vi "WaveAnalysis.vi"() -> (0 "输出图片":picture caption="新图片", 3 "Pixel_in":u8[](array[numeric]) format="%02x", 5 "Gray_in":u8[](array[numeric])=[12, 12, 0, 12, 12, 0, 16, 16, 0, 20, 20, 0, 24, 24, 0, 28, 28, 0, 32, 32, 0, 36, 36, 0, 40, 40, 0, 44, 44, 0, 48, 48, 0, 52, 52, 0, 56, 56, 0, 60, 60, 0, 64, 64, 0, 68, 68, 0, 72, 72, 0, 72, 72, 0, 76, 76, 0, 80, 80, 0, 84, 84, 0, 88, 88, 0, 92, 92, 0, 96, 96, 0, 100, 100, 0, 104, 104, 0, 108, 108, 0, 112, 112, 0, 116, 116, 0, 120, 120, 0, 124, 124, 0, 128, 128, 0, 132, 132, 0, 136, 136, 0, 136, 136, 0, 140, 140, 0, 144, 144, 0, 148, 148, 0, 152, 152, 0, 156, 156, 0, 160, 160, 0, 164, 164, 0, 168, 168, 0, 172, 172, 0, 176, 176, 0, 180, 180, 0, 184, 184, 0, 188, 188, 0, 192, 192, 0, 196, 196, 0, 200, 200, 0, 200, 200, 0, 204, 204, 0, 208, 208, 0, 212, 212, 0, 216, 216, 0, 220, 220, 0, 224, 224, 0, 228, 228, 0, 232, 232, 0, 236, 236, 0, 240, 240, 0, 244, 244, 0, 248, 248, 0, 0, 12, 12, 0, 12, 12, 0, 16, 16, 0, 20, 20, 0, 24, 24, 0, 28, 28, 0, 32, 32, 0, 36, 36, 0, 40, 40, 0, 44, 44, 0, 48, 48, 0, 52, 52, 0, 56, 56, 0, 60, 60, 0, 64, 64, 0, 68, 68, 0, 72, 72, 0, 72, 72, 0, 76, 76, 0, 80, 80, 0, 84, 84, 0, 88, 88, 0, 92, 92, 0, 96, 96, 0, 100, 100, 0, 104, 104, 0, 108, 108, 0, 112, 112, 0, 116, 116, 0, 120, 120, 0, 124, 124, 0, 128, 128, 0, 132, 132, 0, 136, 136, 0, 136, 136, 0, 140, 140, 0, 144, 144, 0, 148, 148, 0, 152, 152, 0, 156, 156, 0, 160, 160, 0, 164, 164, 0, 168, 168, 0, 172, 172, 0, 176, 176, 0, 180, 180, 0, 184, 184, 0, 188, 188, 0, 192, 192, 0, 196, 196, 0, 200, 200, 0, 200, 200, 0, 204, 204, 0, 208, 208, 0, 212, 212, 0, 216, 216, 0, 220, 220, 0, 224, 224, 0, 228, 228, 0, 232, 232, 0, 236, 236, 0, 240, 240, 0, 244, 244, 0, 248, 248] format="%02x")   [LabVIEW 2015]
uses:
  <vilib>/picture/picture.llb/Draw True-Color Pixmap.vi
panel:
  out "像素加粗":picture caption="新图片"
  out "图片缩放":picture caption="新图片"
  in  "像素表路径":path=path "E:/JL-Project/LabView-Project/UPO-Pixel.dat"
  in  "宽度":u32=700
  in  "高度":u32=400
  in  "灰度表路径":path=path "E:/JL-Project/LabView-Project/GrayTable.dat"
  in  "szPixel":u32=3
  in  "m_nGrayScale":u32=64
  in  "m_nCHs":u32=4
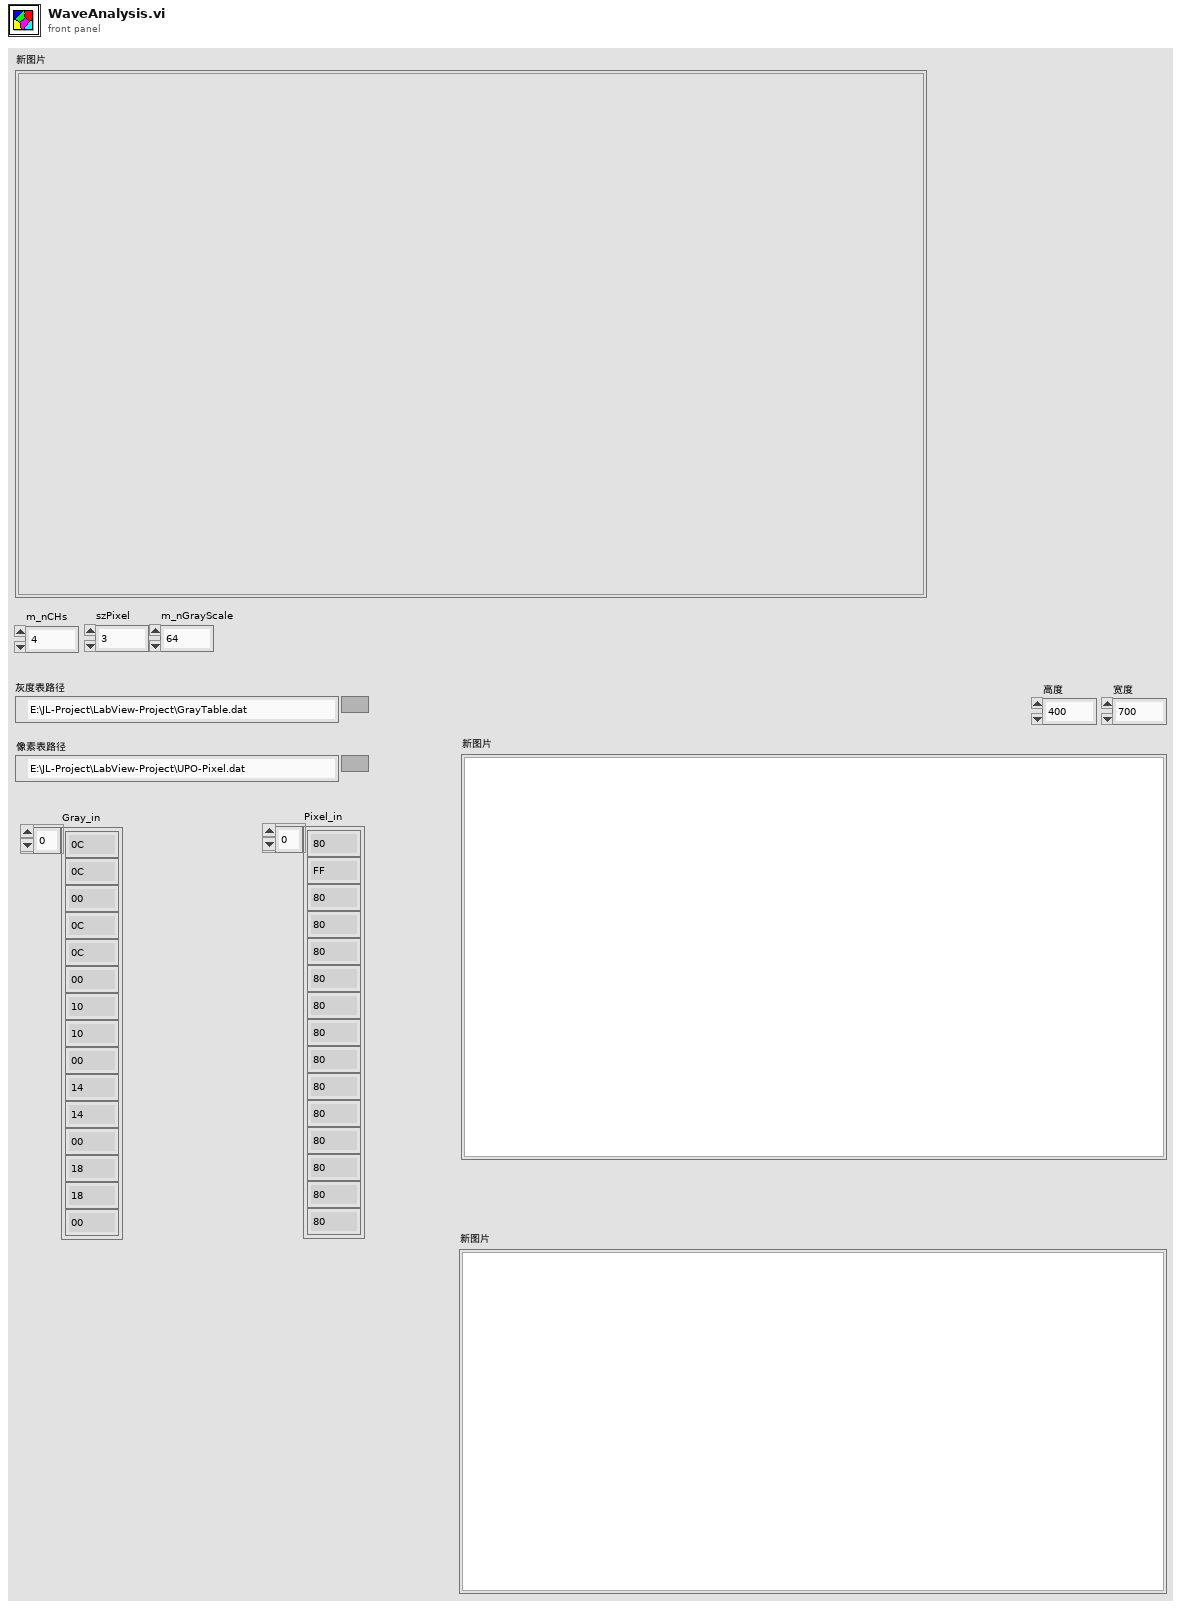
[diagram p1: front panel]
types:
  T1 = enum16{"open", "replace", "create", "open or create", "replace or create", "replace or create with confirmation"}
  T2 = enum16{"big-endian, network order", "native, host order", "little-endian"}
  T3 = typedef "imagedata.ctl" = cluster{"image type":i32, "image depth":i32, "image":u8[], "mask":u8[], "colors":u32[], "Rectangle":cluster{"left":i16, "top":i16, "right":i16, "bottom":i16}}
  T4 = typedef "LVBoundsTypeDef.ctl" = cluster{"Width":u32, "Height":u32}
  T5 = cluster{"left":i16, "top":i16, "right":i16, "bottom":i16}
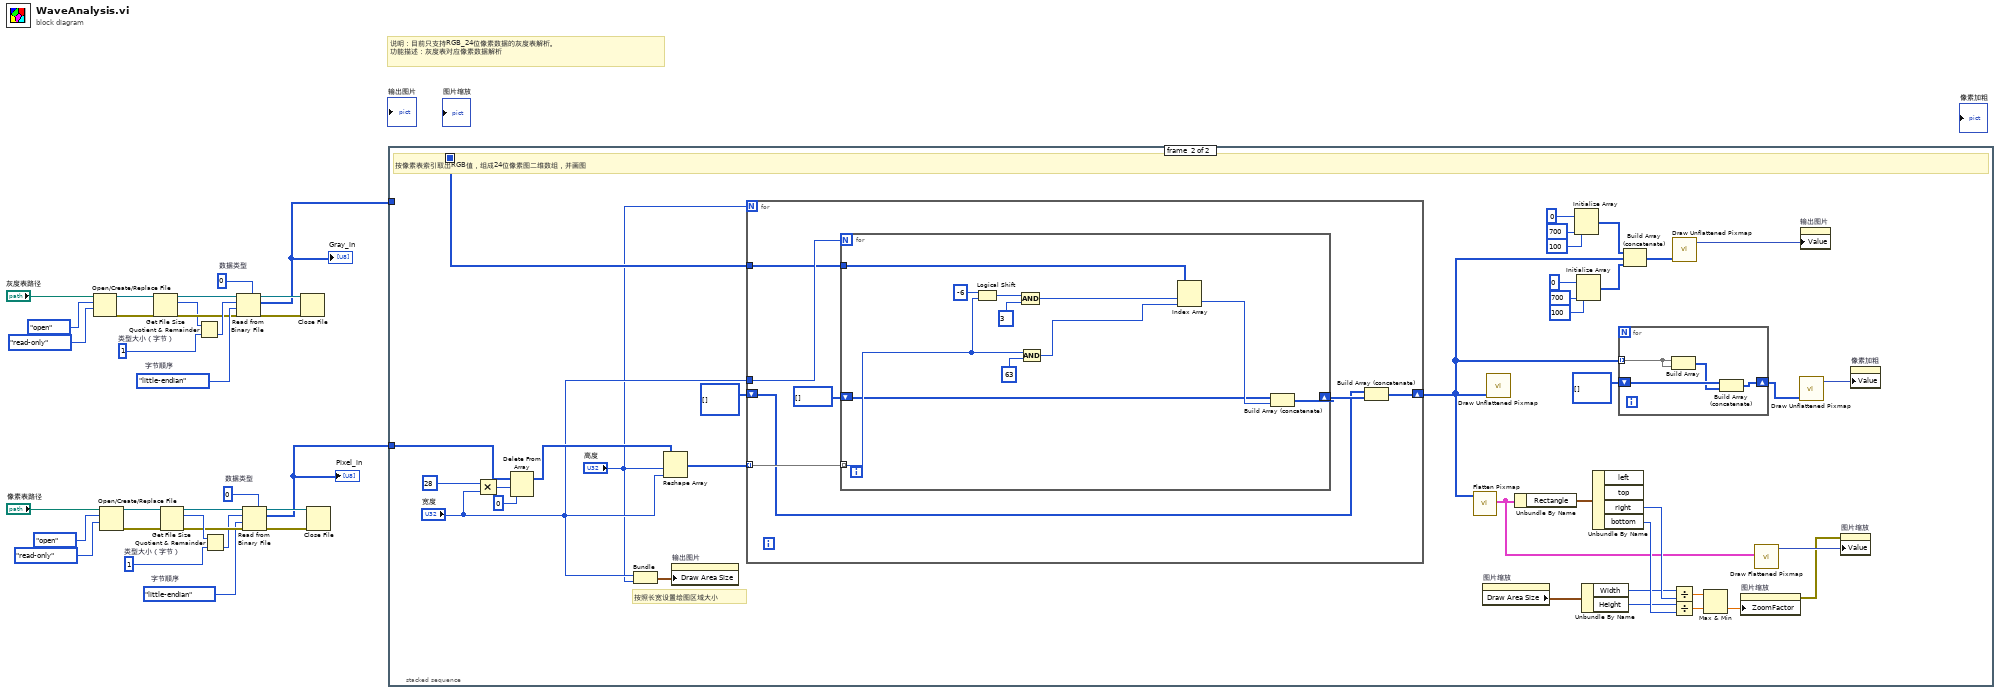
[diagram p0: block diagram]
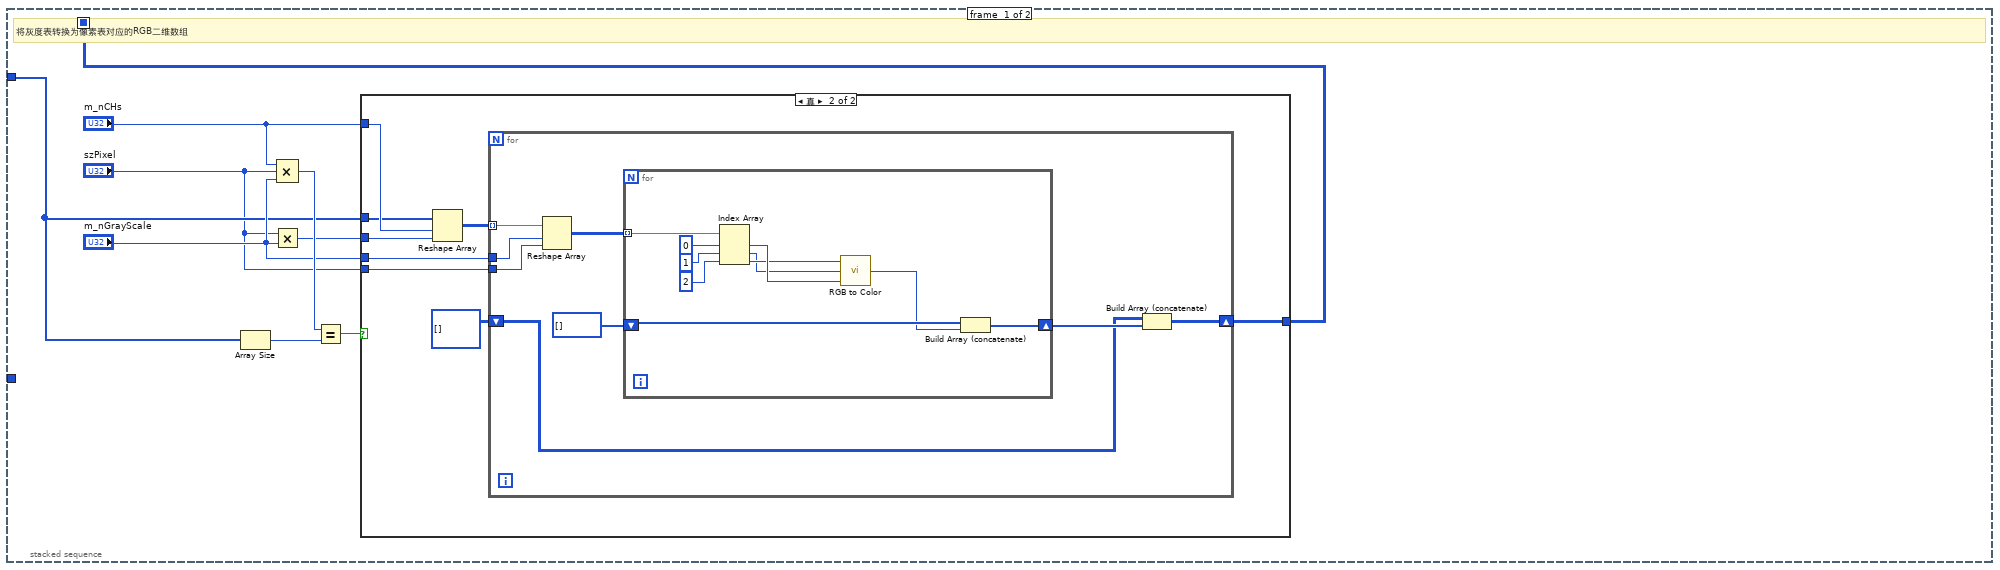
[diagram p2: hidden frame]
diagram:
  w12 = T2."little-endian"  # 字节顺序
  w10 = i64 1  # 类型大小（字节）
  w9 = u8 0  # 数据类型
  w21 = T2."little-endian"  # 字节顺序
  w23 = i64 1  # 类型大小（字节）
  w24 = u8 0  # 数据类型
  # "说明：目前只支持RGB_24位像素数据的灰度表解析。\n功能描述：灰度表对应像素数据解析"
  n1 = Open/Create/Replace File(file path (use dialog)="灰度表路径", operation (0:open)=T1."open", access (0:read/write)=enum16{"read/write", "read-only", "write-only"}."read-only") -> (refnum out=w15:refnum<file>, error out=w14:errorcluster)  [unwired: 3 in, 1 out]
  n2 = Open/Create/Replace File(file path (use dialog)="像素表路径", operation (0:open)=T1."open", access (0:read/write)=enum16{"read/write", "read-only", "write-only"}."read-only") -> (refnum out=w18:refnum<file>, error out=w19:errorcluster)  [unwired: 3 in, 1 out]
  n3 = Get File Size(file=w15, error in=w14) -> (refnum out=w3:refnum<file>, size (in bytes)=w6:i64, 0:w7:errorcluster)
  n4 = Get File Size(file=w18, error in=w19) -> (refnum out=w30:refnum<file>, size (in bytes)=w27:i64, 0:w26:errorcluster)
  n5 = Quotient & Remainder(x=w6, y=w10) -> (floor(x/y)=w11:i64)  [unwired: 1 out]
  n6 = Quotient & Remainder(x=w27, y=w23) -> (floor(x/y)=w22:i64)  [unwired: 1 out]
  n7 = Read from Binary File(5:w9, 8:w7, 9:w12, 10:w11, 11:w3) -> (0:w5:errorcluster, 2:w1:u8[], 3:w4:refnum<file>)  [unwired: 1 in, 1 out]
  "Gray_in" <- w1
  n8 = Read from Binary File(5:w24, 8:w26, 9:w21, 10:w22, 11:w30) -> (0:w28:errorcluster, 2:w2:u8[], 3:w29:refnum<file>)  [unwired: 1 in, 1 out]
  "Pixel_in" <- w2
  n9 = Close File(refnum=w4, error in=w5) -> ()  [unwired: 2 out]
  n10 = Close File(refnum=w29, error in=w28) -> ()  [unwired: 2 out]
  n11 = stacked-sequence {
    seq-local: [w31 _] -> [_ w97]
    tunnel: w1 -> [w33 _]
    tunnel: w2 -> [_ w99]
    frame #0 {
      # "将灰度表转换为像素表对应的RGB二维数组"
      n12 = Array Size(array=w33) -> (size(s)=w38:i32)
      n13 = Multiply(x="szPixel", y="m_nGrayScale") -> (x*y=w35:u32)
      n14 = Compound Arithmetic op=MULTIPLY("m_nCHs", "szPixel", "m_nGrayScale") -> (w39:u32)
      n15 = Equal?(x=w39, y=w38) -> (x = y?=w37:bool)
      n16 = case shown="真" w37 {
        tunnel: "m_nCHs" -> [_ w47]
        tunnel: w33 -> [_ w46]
        tunnel: w35 -> [_ w45]
        tunnel: "szPixel" -> [_ w43]
        tunnel: "m_nGrayScale" -> [_ w42]
        tunnel: [_ w40] -> w31
        frame False {
        }
        frame True {
          n17 = Reshape Array(w46, w47, w45) -> (w44:u8[][])
          n18 = for {
            tunnel: w44 -> [w55] mode=indexing
            tunnel: w43 -> [w53]
            tunnel: w42 -> [w54]
            shift-right: [w49] -> w40
            shift-left: u32[][] [] -> [w50]
            n19 = Reshape Array(w55, w54, w53) -> (w52:u8[][])
            n20 = for {
              tunnel: w52 -> [w63] mode=indexing
              shift-right: [w64] -> w51
              shift-left: u32[] [] -> [w65]
              n21 = Index Array(array=w63, index #1=0 ("索引"), index #2=1 ("索引"), index #3=2 ("索引")) -> (element #1=w59:u8, element #2=w56:u8, element #3=w58:u8)
              n22 = call <vilib>:"RGB to Color.vi"("B"=w59, "G"=w56, "R"=w58) -> ("Color"=w57:u32)
              n23 = Build Array (concatenate)(w65, w57) -> (w64:u32[])
            }
            n24 = Build Array (concatenate)(w50, w51) -> (w49:u32[][])
          }
        }
      }
    }
    frame #1 {
      # "按照长宽设置绘图区域大小"
      # "按像素表索引取出RGB值，组成24位像素图二维数组，并画图"
      n25 = Multiply(x=u32 28, y="宽度") -> (x*y=w101:u32)
      n26 = Delete From Array(array=w99, length=w101, index=0 ("索引")) -> (array with subset deleted=w102:u8[])  [unwired: 1 out]
      n27 = Bundle("宽度"="宽度", "高度"="高度") -> (w95:cluster{"宽度":u32, "高度":u32})  [unwired: 1 in]
      n28 = Reshape Array(w102, "高度", "宽度") -> (w98:u8[][])
      n29 = property on="输出图片" class="Pict"("Draw Area Size"=w95) -> ()  [unwired: 2 in, 2 out]
      n30 = for {
        N: "高度" -> [_]
        tunnel: "宽度" -> [w113]
        tunnel: w98 -> [w112] mode=indexing
        tunnel: w97 -> [w111]
        shift-right: [w108] -> w70
        shift-left: u32[][] [] -> [w107]
        n31 = for {
          N: w113 -> [_]
          tunnel: w112 -> [w118] mode=indexing
          tunnel: w111 -> [w117]
          shift-right: [w115] -> w109
          shift-left: u32[] [] -> [w114]
          n32 = Logical Shift(y=i16 -6, x=w118) -> (x << y=w122:u8)
          n33 = Compound Arithmetic op=AND(w122, u8 3 ("值")) -> (w120:u8)
          n34 = Compound Arithmetic op=AND(w118, u8 63 ("值")) -> (w119:u8)
          n35 = Index Array(array=w117, index (row)=w120, index (col)=w119) -> (element=w116:u32)
          n36 = Build Array (concatenate)(w114, w116) -> (w115:u32[])
        }
        n37 = Build Array (concatenate)(w107, w109) -> (w108:u32[][])
      }
      n38 = call <vilib>:"Flatten Pixmap.vi"("24-bit pixmap"=w70) -> ("image data"=w86:T3)  [unwired: 10 in]
      n39 = property on="图片缩放" class="Pict"() -> ("Draw Area Size"=w82:T4)  [unwired: 2 in, 2 out]
      n40 = call-poly <vilib>:"Draw Unflattened Pixmap.vi"("data (RGB format)"=w70) -> ()  [unwired: 8 in, 1 out]
      n41 = Unbundle By Name(w86) -> ("Rectangle"=w93:T5)
      n42 = Initialize Array(u8 0 ("元素"), 100 ("维数大小"), 700 ("维数大小")) -> (w73:u8[][])
      n43 = Initialize Array(u8 0 ("元素"), 100 ("维数大小"), 700 ("维数大小")) -> (w72:u8[][])
      n44 = Unbundle By Name(w82) -> ("Width"=w81:u32, "Height"=w80:u32)
      n45 = Unbundle By Name(w93) -> ("right"=w92:i16, "bottom"=w90:i16)  [unwired: 2 out]
      n46 = for {
        tunnel: w70 -> [w106] mode=indexing
        shift-right: [w105] -> w68
        shift-left: u32[][] [] -> [w104]
        n47 = Build Array(w106, w106) -> (w103:u32[][])
        n48 = Build Array (concatenate)(w104, w103) -> (w105:u32[][])
      }
      n49 = Build Array (concatenate)(w73, w70, w72) -> (w71:u32[][])
      n50 = call-poly <vilib>:"Draw Unflattened Pixmap.vi"("data (RGB format)"=w71) -> ("new picture"=w67:picture)  [unwired: 8 in]
      n51 = Divide(x=w81, y=w92) -> (x/y=w88:dbl)
      n52 = Divide(x=w80, y=w90) -> (x/y=w87:dbl)
      n53 = Max & Min(x=w88, y=w87) -> (min(x,y)=w85:dbl)  [unwired: 1 out]
      n54 = property on="图片缩放" class="Pict"("ZoomFactor"=w85) -> (error out=w83:errorcluster)  [unwired: 2 in, 1 out]
      n55 = call <vilib>:"Draw Flattened Pixmap.vi"("image data"=w86) -> ("new picture"=w84:picture)  [unwired: 8 in]
      n56 = call-poly <vilib>:"Draw Unflattened Pixmap.vi"("data (RGB format)"=w68) -> ("new picture"=w66:picture)  [unwired: 8 in]
      n57 = property on="输出图片" class="Pict"("Value"=w67) -> ()  [unwired: 2 in, 2 out]
      n58 = property on="图片缩放" class="Pict"(error in=w83, "Value"=w84) -> ()  [unwired: 1 in, 2 out]
      n59 = property on="像素加粗" class="Pict"("Value"=w66) -> ()  [unwired: 2 in, 2 out]
    }
  }
